vi "Snap to top (centered).vi"(1 "Large Rect":T1, 2 "Small Rect":T1) -> (0 "Snapped to top center":T1)   [LabVIEW 2012]
doc: "This VI calculates the position of a snapped-to-top rectangle from the positions of a large rectangle and a smaller one that will be positioned inside."
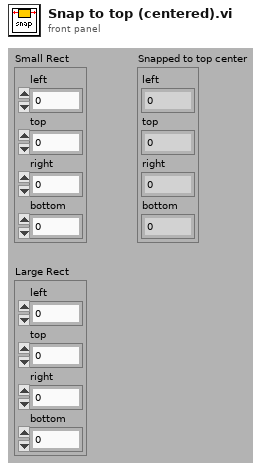
[diagram p1: front panel]
types:
  T1 = cluster{"left":i16, "top":i16, "right":i16, "bottom":i16}
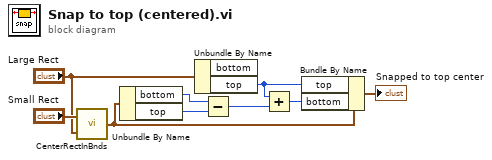
[diagram p0: block diagram]
diagram:
  n1 = call <vilib>:"CenterRectInBnds.vi"("bounds"="Large Rect", "rect"="Small Rect") -> ("centered rect"=w6:T1)
  n2 = Unbundle By Name(w6) -> ("bottom"=w9:i16, "top"=w8:i16)
  n3 = Unbundle By Name("Large Rect") -> ("top"=w4:i16)  [unwired: 1 out]
  n4 = Subtract(x=w9, y=w8) -> (x-y=w7:i16)
  n5 = Add(x=w4, y=w7) -> (x+y=w5:i16)
  n6 = Bundle By Name(cluster=w6, "top"=w4, "bottom"=w5) -> (→"Snapped to top center":T1)
